vi "test protocol version negotiation.vi"(8 "error in (no error)":errorcluster) -> (0 "error out":errorcluster, 3 "body":string)   [LabVIEW 2020, in "MCP Server tests.lvlib"]
doc: "initialize answers with the protocol version the client asked for if the server supports it in the legacy era, otherwise with the version the server prefers: the newest legacy version, 2025-11-25 (it was 2025-06-18 before 2025-11-25 was added)."
uses:
  MCP Server tests.lvlib
  <vilib>/JDP Science/JSONtext/Next JSON Value.vi
  <vilib>/JDP Science/JSONtext/String Subset.vi
  <vilib>/JDP Science/JSONtext/Parsing/Advance past next JSON Value (inlined COPY).vi
  <vilib>/JDP Science/JSONtext/Parsing/Advance past whitespace.vi
  <vilib>/JDP Science/JSONtext/Parsing/Advance past String.vi
  <vilib>/JDP Science/JSONtext/Parsing/Advance past Number.vi
  <vilib>/JDP Science/JSONtext/Parsing/Advance past Line Ending.vi
  <vilib>/JDP Science/JSONtext/Parsing/Parse Full Path or Item Name.vi
  <vilib>/JDP Science/JSONtext/Parsing/Advance past Array.vi
  <vilib>/JDP Science/JSONtext/Parsing/Advance past Object.vi
  <vilib>/JDP Science/JSONtext/support/Error Cluster From Code.vi
  <vilib>/JDP Science/JSONtext/Offset/Find Item Locations by Path.vi
  <vilib>/addons/_JKI Toolkits/Caraya/classes/Test/Test.lvclass
  <vilib>/JDP Science/JSONtext/JSONtext.lvlib
  <vilib>/addons/_JKI Toolkits/Caraya/classes/Assert/Assert.lvclass
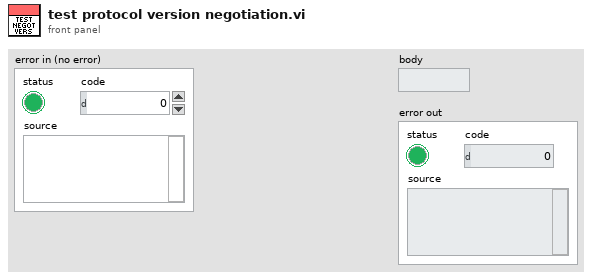
[diagram p1: front panel]
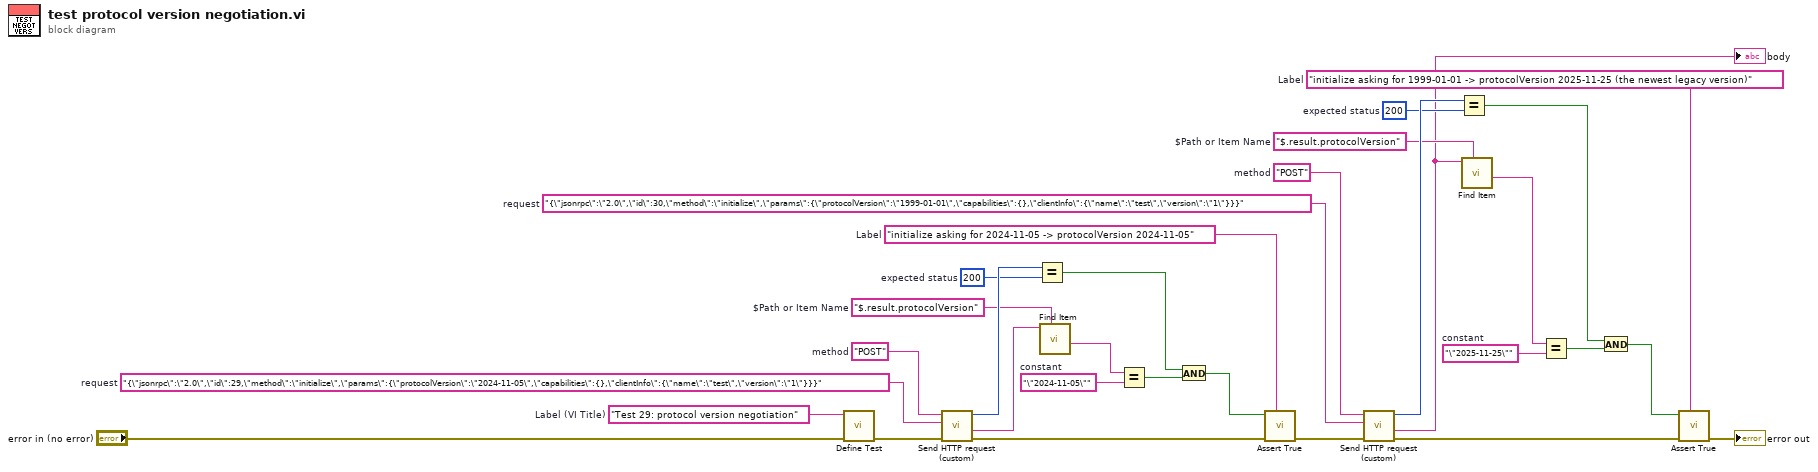
[diagram p0: block diagram]
diagram:
  w3 = "initialize asking for 1999-01-01 -> protocolVersion 2025-11-25 (the newest legacy version)"  # Label
  w8 = "\"2025-11-25\""  # constant
  w10 = "$.result.protocolVersion"  # $Path or Item Name
  w11 = 200  # expected status
  w14 = "{\"jsonrpc\":\"2.0\",\"id\":30,\"method\":\"initialize\",\"params\":{\"protocolVersion\":\"1999-01-01\",\"capabilities\":{},\"clientInfo\":{\"name\":\"test\",\"version\":\"1\"}}}"  # request
  w15 = "POST"  # method
  w16 = "initialize asking for 2024-11-05 -> protocolVersion 2024-11-05"  # Label
  w21 = "\"2024-11-05\""  # constant
  w23 = "$.result.protocolVersion"  # $Path or Item Name
  w25 = 200  # expected status
  w28 = "{\"jsonrpc\":\"2.0\",\"id\":29,\"method\":\"initialize\",\"params\":{\"protocolVersion\":\"2024-11-05\",\"capabilities\":{},\"clientInfo\":{\"name\":\"test\",\"version\":\"1\"}}}"  # request
  w29 = "POST"  # method
  w31 = "Test 29: protocol version negotiation"  # Label (VI Title)
  n1 = call <vilib>:"Define Test.vi"("error in (no error)"="error in (no error)", "Label (VI Title)"=w31) -> ("error out"=w27:errorcluster)  [unwired: 8 in, 1 out]
  n2 = call "Send HTTP request (custom).vi"("error in (no error)"=w27, "request"=w28, "method"=w29) -> ("error out"=w17:errorcluster, "response"=w24:string, "status code"=w26:i32)  [unwired: 5 in, 1 out]
  n3 = Equal?(x=w26, y=w25) -> (x = y?=w20:bool)
  n4 = call <vilib>:"Find Item.vi"("$Path or Item Name"=w23, "JSON"=w24) -> ("<JSON>"=w22:string)  [unwired: 6 in, 3 out]
  n5 = Equal?(x=w22, y=w21) -> (x = y?=w19:bool)
  n6 = And(x=w20, y=w19) -> (x .and. y?=w18:bool)
  n7 = call <vilib>:"Assert True.vi"("Label"=w16, "error in (no error)"=w17, "True?"=w18) -> ("error out"=w13:errorcluster)  [unwired: 7 in, 1 out]
  n8 = call "Send HTTP request (custom).vi"("error in (no error)"=w13, "request"=w14, "method"=w15) -> ("error out"=w4:errorcluster, "response"=w2:string, "status code"=w12:i32)  [unwired: 5 in, 1 out]
  "body" <- w2
  n9 = Equal?(x=w12, y=w11) -> (x = y?=w7:bool)
  n10 = call <vilib>:"Find Item.vi"("$Path or Item Name"=w10, "JSON"=w2) -> ("<JSON>"=w9:string)  [unwired: 6 in, 3 out]
  n11 = Equal?(x=w9, y=w8) -> (x = y?=w6:bool)
  n12 = And(x=w7, y=w6) -> (x .and. y?=w5:bool)
  n13 = call <vilib>:"Assert True.vi"("Label"=w3, "error in (no error)"=w4, "True?"=w5) -> ("error out"=→"error out":errorcluster)  [unwired: 7 in, 1 out]
